vi "DE10_DAQ.vi"() -> ()   [LabVIEW 2014]
uses:
  Control 1.ctl
  <vilib>/Analysis/baseanly.llb/Mean (DBL).vi
  <vilib>/Analysis/NI_AALBase.lvlib
panel:
  in  "IP Address":string="142.90.140.191"
  out "Selected Analog values":dbl(graph)
  out "Logic Mask":T1={"Up"=FALSE, "Down"=TRUE, "Left"=TRUE, "Right"=TRUE, "Halo"=FALSE, "Density"=FALSE, "Total"=FALSE, "HV"=FALSE, "|L-R|"=FALSE, "|U-D|"=TRUE, "|Den-Tot|"=TRUE, "Sum/Tot"=TRUE, "Tot-Sum"=FALSE, "T1 Vac"=FALSE, "T2 Sum"=FALSE, "TNF Sum"=FALSE}
  out "Digital Input":bool[](array[boolean])
  out "Relay Contact output":bool[](array[boolean])
  in  "Analog Parameter Threshold Setting:":string[][](table) caption="Analog Readback values"
  in  "Update Threshold":bool
  in  "Mask Register":T2={"Up"=FALSE, "Down"=TRUE, "Left"=TRUE, "Right"=TRUE, "Halo"=FALSE, "Density"=FALSE, "Total"=FALSE, "HV"=FALSE, "|L-R|"=FALSE, "|U-D|"=TRUE, "|Den-total|"=TRUE, "Sum/Tot"=TRUE, "Tot-Sum"=FALSE, "T1 Vac"=FALSE, "T2 Sum"=FALSE, "TNF Sum"=FALSE}
  in  "Update PCA gain":bool
  in  "Ch7":enum32{"G0", "G1", "G2", "G3"}(radio)
  in  "Ch6":enum32{"G0", "G1", "G2", "G3"}(radio)
  in  "Ch5":enum32{"G0", "G1", "G2", "G3"}(radio)
  in  "Ch4":enum32{"G0", "G1", "G2", "G3"}(radio)
  in  "Ch3":enum32{"G0", "G1", "G2", "G3"}(radio)
  in  "Ch2":enum32{"G0", "G1", "G2", "G3"}(radio)
  in  "Ch1":enum32{"G0", "G1", "G2", "G3"}(radio)
  in  "Ch0":enum32{"G0", "G1", "G2", "G3"}(radio)
  in  "Control Register":T3={"Output Relay"=FALSE, "Not in use"=TRUE, "Ena temp"=TRUE, "PCA Cal"=FALSE}
  in  "flash2conf":bool
  in  "conf2flash":bool
  out "Analog input channel readback - high precision:":string[][](table) caption="Analog Readback values"
  out "Threshold values:":string[][](table) caption="Analog Readback values"
  out "Analog Parameter and Threshold value readback:":T4 caption="Analog Readback values"
  out "Interlock Status":bool[](array[boolean])
  out "Control Register":bool[](array[boolean])
  out "Temperature":dbl(graph)
  out "sFIFO Words":i32=1024
  out "Display channel":u16
  out "Avg (mV)":dbl format="%#_4g"
  out "RMS (mV)":dbl format="%#_4g"
  in  "Waveform\nChannel":T5(radio)
  out "MB Firmware ver:":string="FPGA_VER?"
  out "FPGA ver:":string="FPGA_VER?"
  in  "Enable waveform Acq":bool
  out "Fast FIFO( waveform from selected channel)":dbl[](graph)
  in  "Reg name":string
  out "Read back Value":i32 format="%x"
  in  "Read":bool
  in  "Value to write":i32
  in  "Write":bool
  in  "stop":bool
  in  "PORT":u16=2022
  out "error out":errorcluster
  # "Notes: \n1.) Noise p-p value: measrued on Dec.2,2018:\n40 pA for HG, 10 nA for LG;\n2.) Trancation error gives -0.07 uA for Analog value readback;\nLast updated: January 8,2019 \n3.)Mask bit: check means \"paticipation\""
  # "PCA gain selection:"
  # "Conf EEPROM operation"
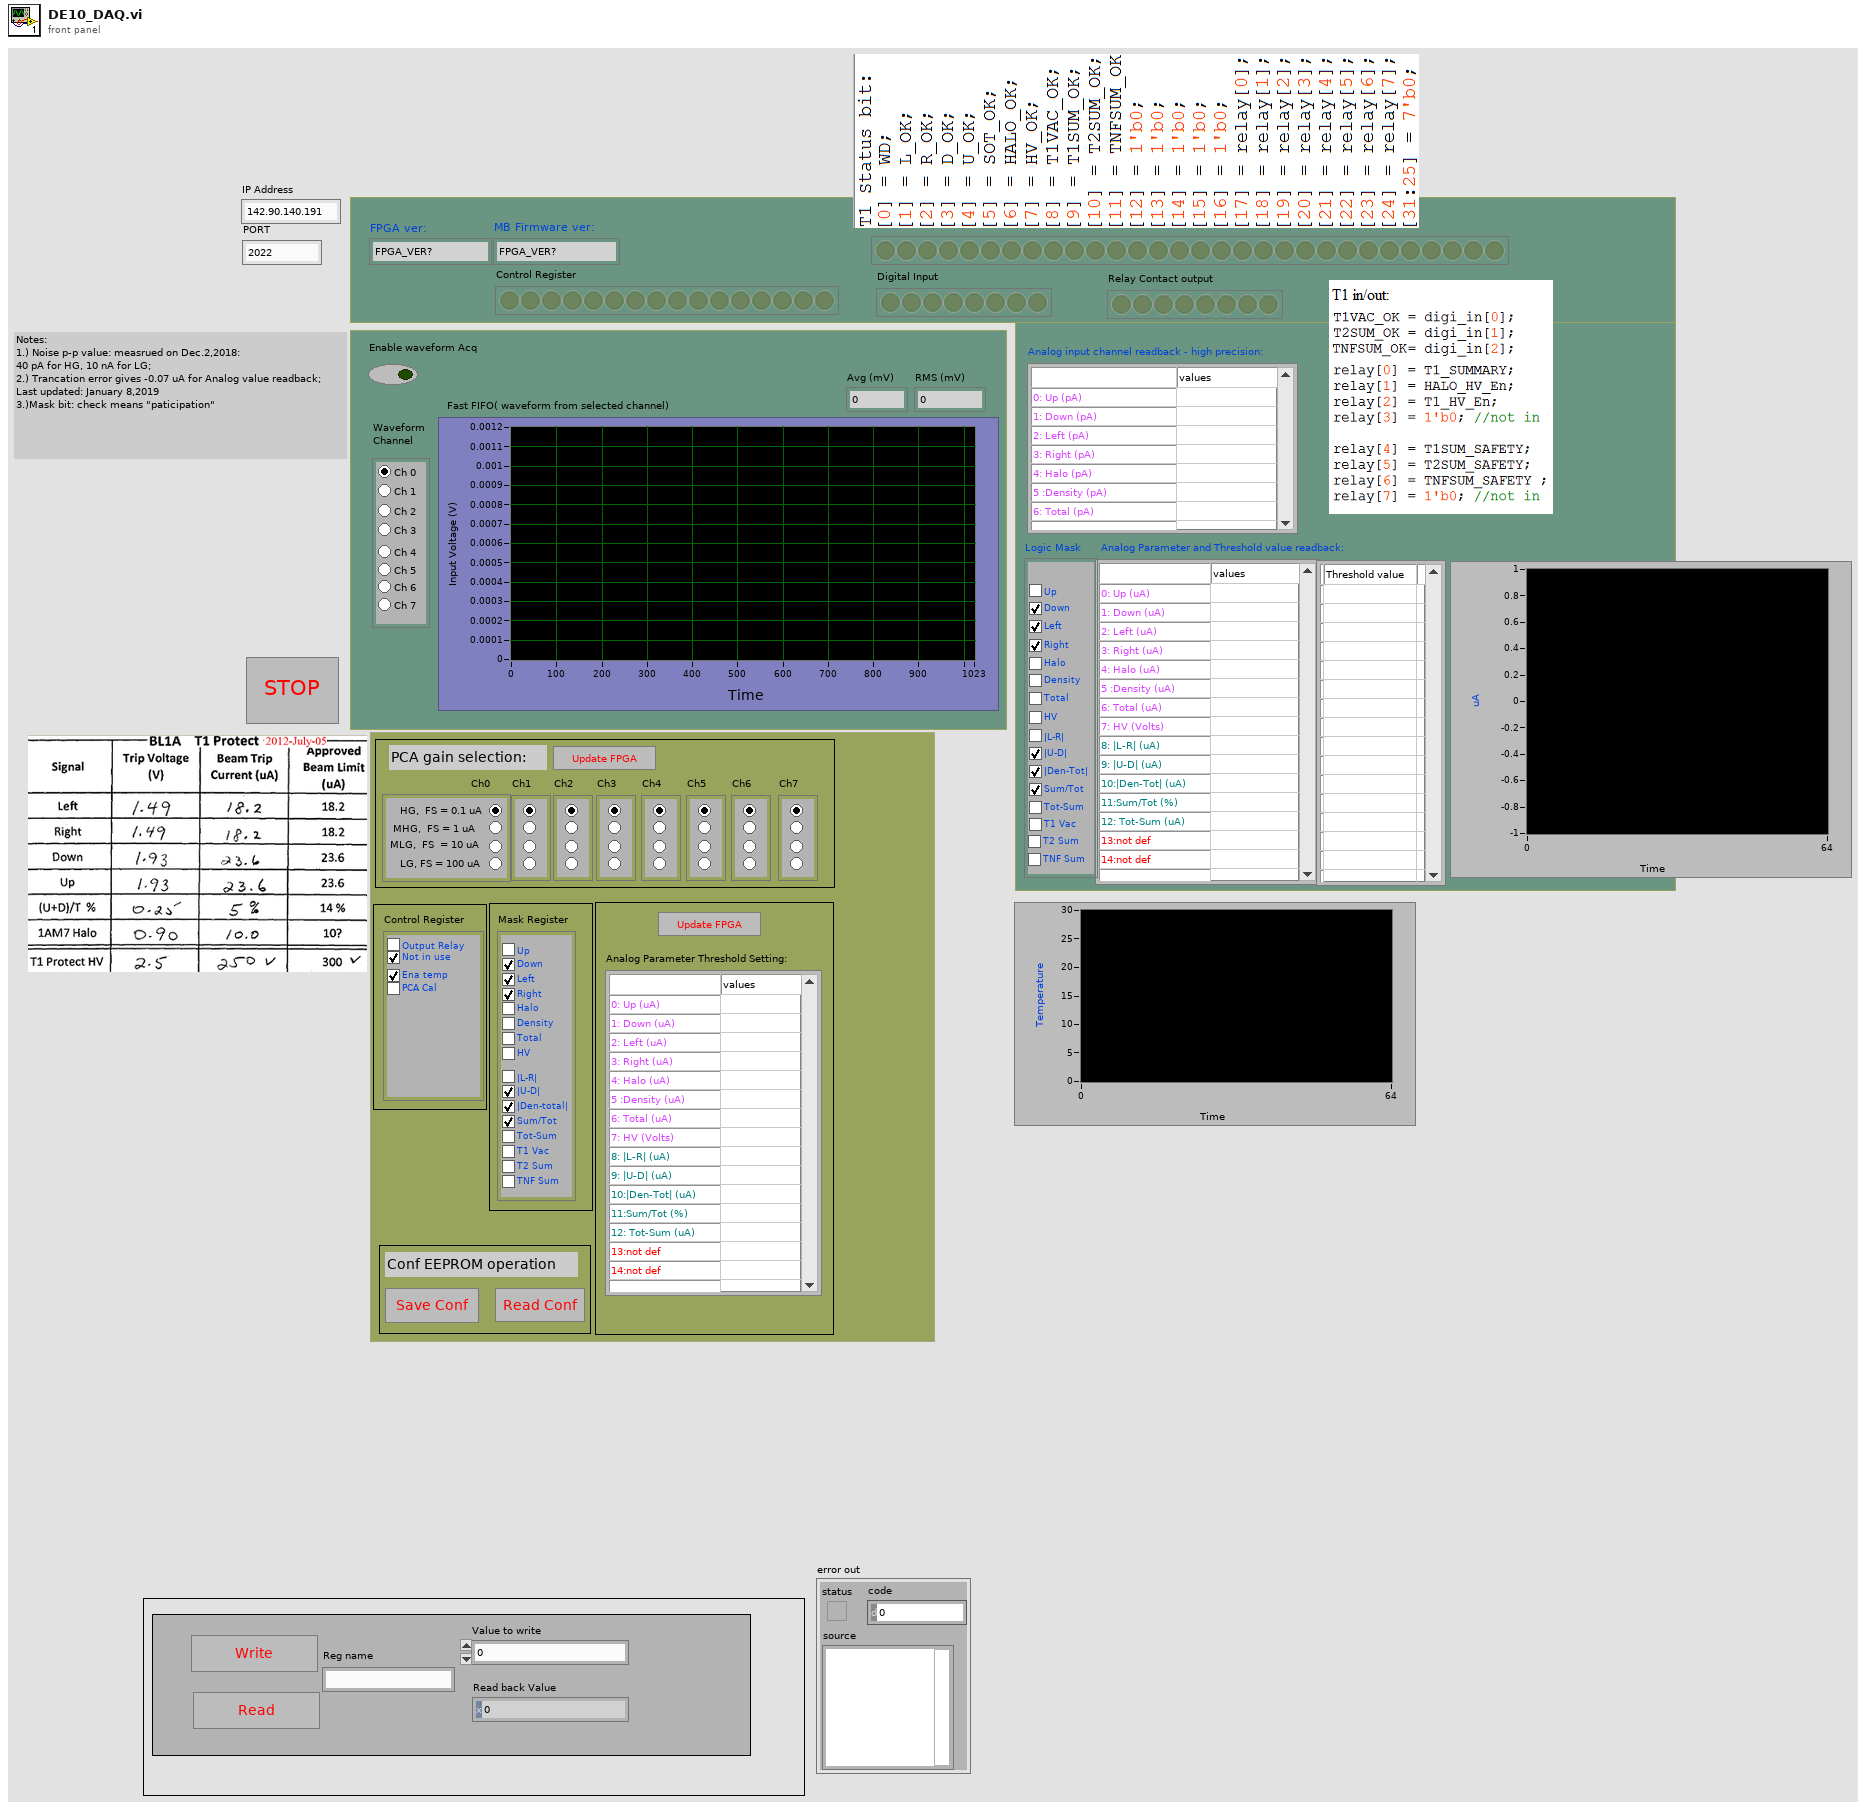
[diagram p1: front panel]
types:
  T1 = cluster{"Up":bool, "Down":bool, "Left":bool, "Right":bool, "Halo":bool, "Density":bool, "Total":bool, "HV":bool, "|L-R|":bool, "|U-D|":bool, "|Den-Tot|":bool, "Sum/Tot":bool, "Tot-Sum":bool, "T1 Vac":bool, "T2 Sum":bool, "TNF Sum":bool}
  T2 = cluster{"Up":bool, "Down":bool, "Left":bool, "Right":bool, "Halo":bool, "Density":bool, "Total":bool, "HV":bool, "|L-R|":bool, "|U-D|":bool, "|Den-total|":bool, "Sum/Tot":bool, "Tot-Sum":bool, "T1 Vac":bool, "T2 Sum":bool, "TNF Sum":bool}
  T3 = cluster{"Output Relay":bool, "Not in use":bool, "Ena temp":bool, "PCA Cal":bool}
  T4 = typedef "Control 1.ctl" = string[][]
  T5 = enum32{"Ch 0", "Ch 1", "Ch 2", "Ch 3", "Ch 4", "Ch 5", "Ch 6", "Ch 7"}
  T6 = cluster{bool, bool, bool, bool, bool, bool, bool, bool, bool, bool, bool, bool, bool, bool, bool, bool}
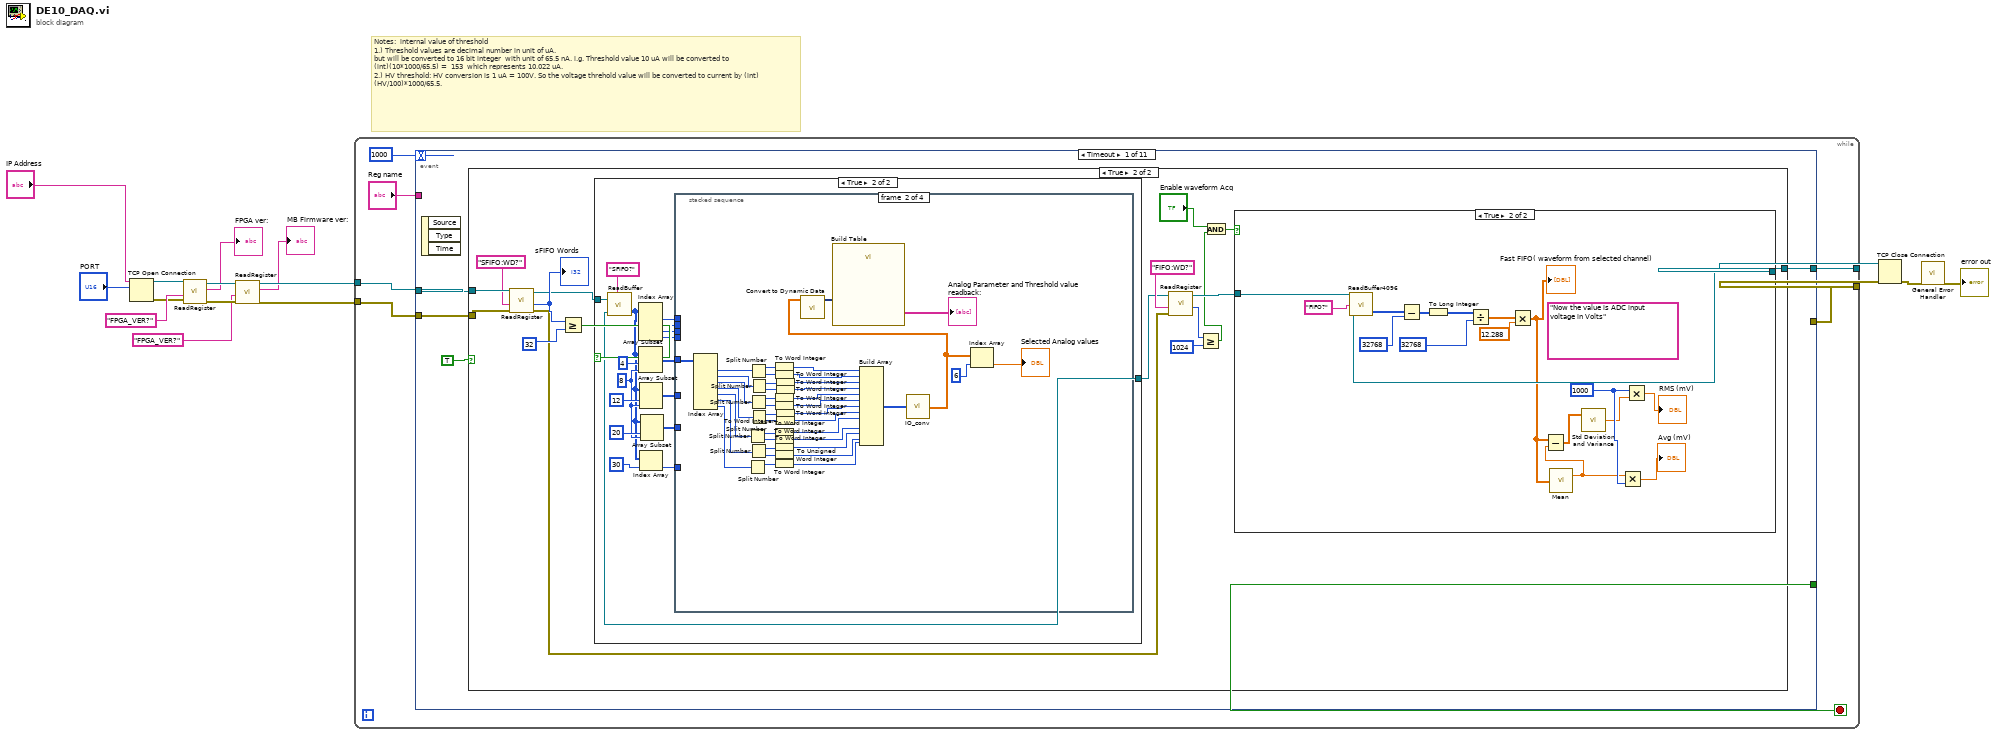
[diagram p0: block diagram]
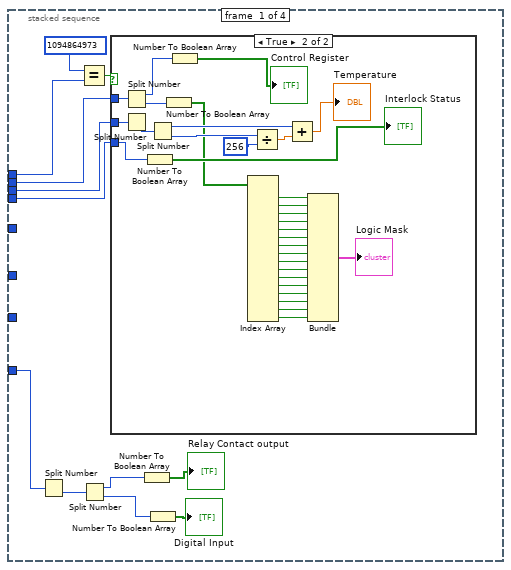
[diagram p4: hidden frame]
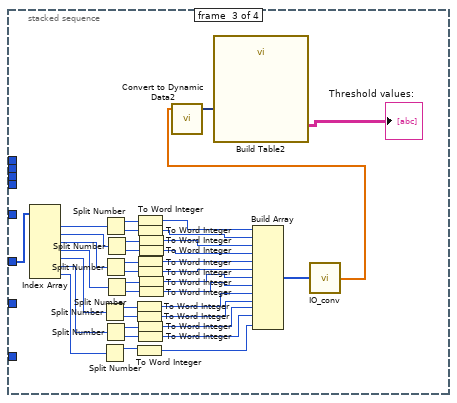
[diagram p6: hidden frame]
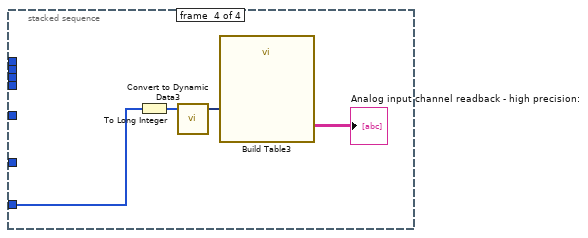
[diagram p7: hidden frame]
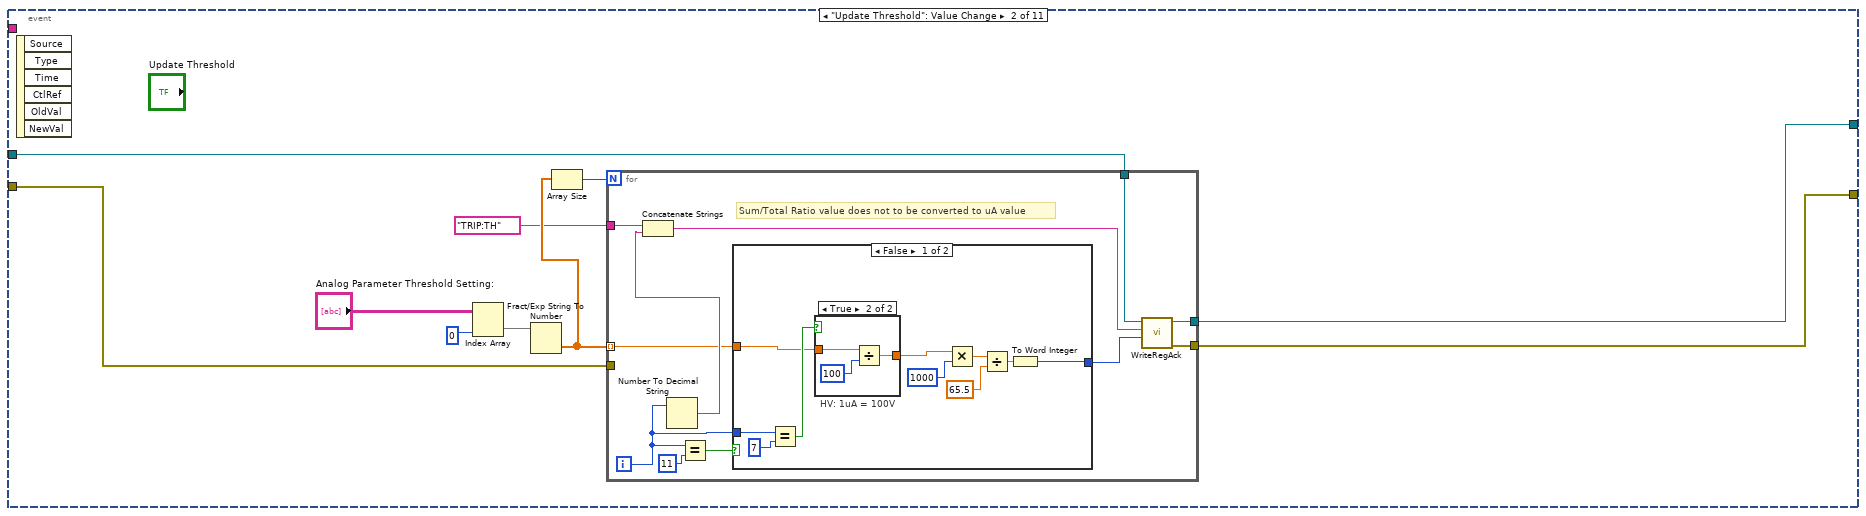
[diagram p9: hidden frame]
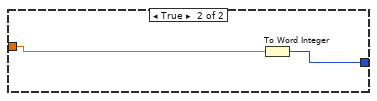
[diagram p11: hidden frame]
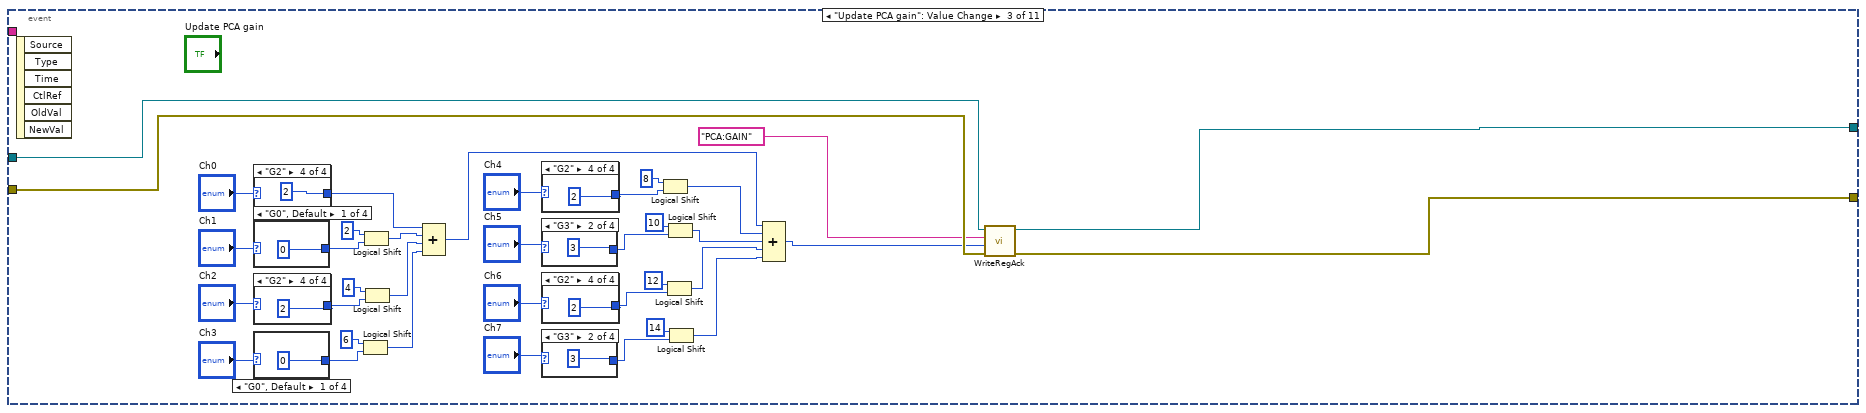
[diagram p12: hidden frame]
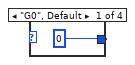
[diagram p13: hidden frame]
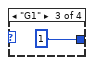
[diagram p14: hidden frame]
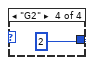
[diagram p15: hidden frame]
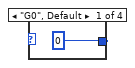
[diagram p16: hidden frame]
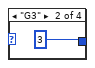
[diagram p17: hidden frame]
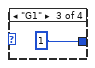
[diagram p18: hidden frame]
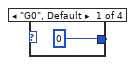
[diagram p19: hidden frame]
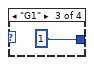
[diagram p20: hidden frame]
diagram:
  # "Notes:  internal value of threshold \n1.) Threshold values are decimal number in unit of uA.\nbut will be converted to 16 bit integer  with unit of 65.5 nA. i.g. Threshold value 10 uA will be converted to (int)(10*1000/65.5) =  153  which represents 10.022 uA. \n2.) HV threshold: HV conversion is 1 uA = 100V. So the voltage threhold value will be converted to current by (int) (HV/100)*1000/65.5."
  n1 = TCP Open Connection(address="IP Address", remote port or service name="PORT") -> (connection ID=w11:refnum<k5>, error out=w7:errorcluster)  [unwired: 3 in]
  n2 = call "ReadRegister.vi"("error in"=w7, "string in"="FPGA_VER?", "connection ID in"=w11) -> ("error out"=w6:errorcluster, "string out"=→"FPGA ver:":string, "connection ID out"=w10:refnum<k5>)  [unwired: 2 in, 2 out]
  n3 = call "ReadRegister.vi"("error in"=w6, "string in"="FPGA_VER?", "connection ID in"=w10) -> ("error out"=w5:errorcluster, "string out"=→"MB Firmware ver:":string, "connection ID out"=w9:refnum<k5>)  [unwired: 2 in, 2 out]
  n4 = while {
    tunnel: [w23] -> w15
    tunnel: [w22] -> w14
    tunnel: w9 -> [w18]
    tunnel: w5 -> [w17]
    stop <- w21 stop-if-true
    n5 = event shown="[0] Timeout" {
      selector: _ -> [_ _ _ _ _ _ _ _ _ _ _]
      dyn-events: _ -> [_ _ _ _ _ _ _ _ _ _ _]
      timeout: 1000 -> [_ _ _ _ _ _ _ _ _ _ _]
      tunnel: w18 -> [w26 w210 w249 w318 w330 w334 w361 w375 w381 w384 w473]
      tunnel: [w27 w208 w247 w316 w327 w333 w356 _ w379 _ w473] -> w23
      tunnel: w17 -> [w25 w209 w248 w317 w329 w331 w360 w373 w377 w385 w472]
      tunnel: [_ w207 w246 w315 w328 w332 w357 w372 w378 _ w472] -> w22
      tunnel: [_ _ _ _ _ _ _ _ _ _ "stop"] -> w21
      tunnel: "Reg name" -> [_ _ _ w313 _ _ _ _ _ _ _]
      tunnel: [_ _ _ _ _ _ _ w371 _ _ _] -> _
      event Timeout {
        n6 = event-data() -> ()  [unwired: 1 in, 3 out]
        n7 = case shown="True" TRUE {
          tunnel: [w28 w45] -> w27
          tunnel: w26 -> [w28 w40]
          tunnel: w25 -> [_ w39]
          frame False {
          }
          frame True {
            n8 = call "ReadRegister.vi"("error in"=w39, "string in"="SFIFO:WD?", "connection ID in"=w40) -> ("error out"=w32:errorcluster, "number out"=w36:i32, "connection ID out"=w34:refnum<k5>)  [unwired: 2 in, 2 out]
            "sFIFO Words" <- w36
            n9 = Greater Or Equal?(x=w36, y=32) -> (x >= y?=w35:bool)
            n10 = case shown="True" w35 {
              tunnel: w34 -> [w46 w62]
              tunnel: [w46 w57] -> w33
              frame False {
              }
              frame True {
                w51 = 8
                n11 = call "ReadBuffer.vi"("string in"="SFIFO?", "connection ID in"=w62) -> ("FIFO32_data"=w48:u32[], "connection ID out"=w57:refnum<k5>)  [unwired: 2 in]
                n12 = Index Array(array=w48) -> (element #1=w61:u32, element #2=w60:u32, element #3=w59:u32, element #4=w58:u32)  [unwired: 4 in]
                n13 = Array Subset(array=w48, index=4, length=w51) -> (w55:u32[])
                n14 = Array Subset(array=w48, index=12, length=w51) -> (w54:u32[])
                n15 = Index Array(array=w48, index=30) -> (element=w47:u32)
                n16 = Array Subset(array=w48, index=20, length=w51) -> (w50:u32[])
                n17 = stacked-sequence {
                  tunnel: w61 -> [w74 _ _ _]
                  tunnel: w60 -> [w72 _ _ _]
                  tunnel: w59 -> [w71 _ _ _]
                  tunnel: w58 -> [w70 _ _ _]
                  tunnel: w55 -> [_ w146 _ _]
                  tunnel: w54 -> [_ _ w151 _]
                  tunnel: w50 -> [_ _ _ w185]
                  tunnel: w47 -> [w69 _ _ _]
                  frame #0 {
                    n18 = Split Number(x=w69) -> (lo(x)=w68:u16)  [unwired: 1 out]
                    n19 = Equal?(x=u32 1094864973, y=w74) -> (x = y?=w73:bool)
                    n20 = Split Number(x=w68) -> (hi(x)=w66:u8, lo(x)=w65:u8)
                    n21 = case shown="True" w73 {
                      tunnel: w72 -> [_ w106]
                      tunnel: w71 -> [_ w99]
                      tunnel: w70 -> [_ w95]
                      frame False {
                      }
                      frame True {
                        n22 = Split Number(x=w106) -> (hi(x)=w101:u16, lo(x)=w105:u16)
                        n23 = Split Number(x=w99) -> (lo(x)=w98:u16)  [unwired: 1 out]
                        n24 = Number To Boolean Array(number=w95) -> (Boolean array=→"Interlock Status":bool[])
                        n25 = Split Number(x=w98) -> (hi(x)=w96:u8, lo(x)=w97:u8)
                        n26 = Number To Boolean Array(number=w105) -> (Boolean array=w76:bool[])
                        n27 = Number To Boolean Array(number=w101) -> (Boolean array=→"Control Register":bool[])
                        n28 = Index Array(array=w76) -> (element #1=w77:bool, element #2=w78:bool, element #3=w79:bool, element #4=w80:bool, element #5=w81:bool, element #6=w82:bool, element #7=w83:bool, element #8=w84:bool, element #9=w85:bool, element #10=w86:bool, element #11=w87:bool, element #12=w88:bool, element #13=w89:bool, element #14=w90:bool, element #15=w91:bool, element #16=w92:bool)  [unwired: 16 in]
                        n29 = Divide(x=w97, y=256) -> (x/y=w103:dbl)
                        n30 = Add(x=w96, y=w103) -> (x+y=→"Temperature":dbl)
                        n31 = Bundle(w77, w78, w79, w80, w81, w82, w83, w84, w85, w86, w87, w88, w89, w90, w91, w92) -> (→"Logic Mask":T6)  [unwired: 1 in]
                      }
                    }
                    n32 = Number To Boolean Array(number=w66) -> (Boolean array=→"Relay Contact output":bool[])
                    n33 = Number To Boolean Array(number=w65) -> (Boolean array=→"Digital Input":bool[])
                  }
                  frame #1 {
                    n34 = Index Array(array=w146) -> (element #1=w145:u32, element #2=w136:u32, element #3=w135:u32, element #4=w134:u32, element #5=w129:u32, element #6=w128:u32, element #7=w127:u32)  [unwired: 7 in]
                    n35 = Split Number(x=w129) -> (hi(x)=w133:u16, lo(x)=w132:u16)
                    n36 = Split Number(x=w127) -> (hi(x)=w111:u16)  [unwired: 1 out]
                    n37 = Split Number(x=w145) -> (hi(x)=w144:u16, lo(x)=w143:u16)
                    n38 = Split Number(x=w135) -> (hi(x)=w140:u16, lo(x)=w139:u16)
                    n39 = Split Number(x=w128) -> (hi(x)=w131:u16, lo(x)=w130:u16)
                    n40 = Split Number(x=w136) -> (hi(x)=w142:u16, lo(x)=w141:u16)
                    n41 = Split Number(x=w134) -> (hi(x)=w138:u16, lo(x)=w137:u16)
                    n42 = To Word Integer(number=w133) -> (16bit integer=w118:i16)
                    n43 = To Word Integer(number=w132) -> (16bit integer=w117:i16)
                    n44 = To Word Integer(number=w111) -> (16bit integer=w112:i16)
                    n45 = To Word Integer(number=w144) -> (16bit integer=w126:i16)
                    n46 = To Word Integer(number=w143) -> (16bit integer=w119:i16)
                    n47 = To Word Integer(number=w140) -> (16bit integer=w123:i16)
                    n48 = To Word Integer(number=w139) -> (16bit integer=w122:i16)
                    n49 = To Word Integer(number=w131) -> (16bit integer=w116:i16)
                    n50 = To Unsigned Word Integer(number=w130) -> (unsigned 16bit integer=w115:u16)
                    n51 = To Word Integer(number=w142) -> (16bit integer=w125:i16)
                    n52 = To Word Integer(number=w141) -> (16bit integer=w124:i16)
                    n53 = To Word Integer(number=w138) -> (16bit integer=w121:i16)
                    n54 = To Word Integer(number=w137) -> (16bit integer=w120:i16)
                    n55 = Build Array(w126, w119, w125, w124, w123, w122, w121, w120, w118, w117, w116, w115, w112) -> (w110:u16[])
                    n56 = call "IO_conv.vi"("input"=w110) -> ("output"=w109:dbl[])
                    n57 = call "Convert to Dynamic Data"("Array"=w109) -> ("Dynamic Data Type"=w114:dynamicdata)  [unwired: 3 in]
                    n58 = call "Build Table"("Signals"=w114) -> ("Table"=→"Analog Parameter and Threshold value readback:":string[][])  [unwired: 9 in, 1 out]
                    n59 = Index Array(array=w109, index=6) -> (element=→"Selected Analog values":dbl)
                  }
                  frame #2 {
                    n60 = Index Array(array=w151) -> (element #1=w183:u32, element #2=w174:u32, element #3=w173:u32, element #4=w172:u32, element #5=w167:u32, element #6=w166:u32, element #7=w165:u32)  [unwired: 7 in]
                    n61 = Split Number(x=w167) -> (hi(x)=w171:u16, lo(x)=w170:u16)
                    n62 = Split Number(x=w165) -> (hi(x)=w149:u16)  [unwired: 1 out]
                    n63 = Split Number(x=w183) -> (hi(x)=w182:u16, lo(x)=w181:u16)
                    n64 = Split Number(x=w173) -> (hi(x)=w178:u16, lo(x)=w177:u16)
                    n65 = Split Number(x=w166) -> (hi(x)=w169:u16, lo(x)=w168:u16)
                    n66 = Split Number(x=w174) -> (hi(x)=w180:u16, lo(x)=w179:u16)
                    n67 = Split Number(x=w172) -> (hi(x)=w176:u16, lo(x)=w175:u16)
                    n68 = To Word Integer(number=w171) -> (16bit integer=w156:i16)
                    n69 = To Word Integer(number=w170) -> (16bit integer=w155:i16)
                    n70 = To Word Integer(number=w149) -> (16bit integer=w152:i16)
                    n71 = To Word Integer(number=w182) -> (16bit integer=w164:i16)
                    n72 = To Word Integer(number=w181) -> (16bit integer=w157:i16)
                    n73 = To Word Integer(number=w178) -> (16bit integer=w161:i16)
                    n74 = To Word Integer(number=w177) -> (16bit integer=w160:i16)
                    n75 = To Word Integer(number=w169) -> (16bit integer=w154:i16)
                    n76 = To Word Integer(number=w168) -> (16bit integer=w153:i16)
                    n77 = To Word Integer(number=w180) -> (16bit integer=w163:i16)
                    n78 = To Word Integer(number=w179) -> (16bit integer=w162:i16)
                    n79 = To Word Integer(number=w176) -> (16bit integer=w159:i16)
                    n80 = To Word Integer(number=w175) -> (16bit integer=w158:i16)
                    n81 = Build Array(w164, w157, w163, w162, w161, w160, w159, w158, w156, w155, w154, w153, w152) -> (w148:i16[])
                    n82 = call "IO_conv.vi"("input"=w148) -> ("output"=w147:dbl[])
                    n83 = call "Convert to Dynamic Data2"("Array"=w147) -> ("Dynamic Data Type"=w184:dynamicdata)  [unwired: 3 in]
                    n84 = call "Build Table2"("Signals"=w184) -> ("Table"=→"Threshold values:":string[][])  [unwired: 9 in, 1 out]
                  }
                  frame #3 {
                    n85 = To Long Integer(number=w185) -> (32bit integer=w186:i32[])
                    n86 = call "Convert to Dynamic Data3"("Array"=w186) -> ("Dynamic Data Type"=w188:dynamicdata)  [unwired: 3 in]
                    n87 = call "Build Table3"("Signals"=w188) -> ("Table"=→"Analog input channel readback - high precision:":string[][])  [unwired: 9 in, 1 out]
                  }
                }
              }
            }
            n88 = call "ReadRegister.vi"("error in"=w32, "string in"="FIFO:WD?", "connection ID in"=w33) -> ("number out"=w41:i32, "connection ID out"=w44:refnum<k5>)  [unwired: 2 in, 3 out]
            n89 = Greater Or Equal?(x=w41, y=1024) -> (x >= y?=w29:bool)
            n90 = And(x="Enable waveform Acq", y=w29) -> (x .and. y?=w30:bool)
            n91 = case shown="True" w30 {
              tunnel: [w189 w206] -> w45
              tunnel: w44 -> [w189 w205]
              frame False {
              }
              frame True {
                w195 = 1000
                (unwired) "Now the value is ADC input voltage in Volts"
                n92 = call "ReadBuffer4096.vi"("string in"="FIFO?", "connection ID in"=w205) -> ("FIFO32_data"=w200:u32[], "connection ID out"=w206:refnum<k5>)  [unwired: 2 in]
                n93 = Subtract(x=w200, y=32768) -> (x-y=w197:u32[])
                n94 = To Long Integer(number=w197) -> (32bit integer=w198:i32[])
                n95 = Divide(x=w198, y=32768) -> (x/y=w199:dbl[])
                n96 = Multiply(x=w199, y=12.288) -> (x*y=w191:dbl[])
                "Fast FIFO( waveform from selected channel)" <- w191
                n97 = call-poly <vilib>:"Mean.vi"("X"=w191) -> ("mean"=w192:dbl)  [unwired: 1 out]
                n98 = Subtract(x=w191, y=w192) -> (x-y=w190:dbl[])
                n99 = call <vilib>:"Std Deviation and Variance.vi"("X"=w190) -> ("standard deviation"=w194:dbl)  [unwired: 1 in, 2 out]
                n100 = Multiply(x=w192, y=w195) -> (x*y=→"Avg (mV)":dbl)
                n101 = Multiply(x=w195, y=w194) -> (x*y=→"RMS (mV)":dbl)
              }
            }
          }
        }
      }
      event "Update Threshold": Value Change {
        n102 = event-data() -> ()  [unwired: 1 in, 6 out]
        n103 = Index Array(array="Analog Parameter Threshold Setting:", index (col)=0) -> (element=w215:string[])  [unwired: 1 in]
        n104 = Fract/Exp String To Number(string=w215) -> (number=w212:dbl[])  [unwired: 3 in, 1 out]
        n105 = Array Size(array=w212) -> (size(s)=w213:i32)
        n106 = for {
          N: w213 -> [_]
          tunnel: w212 -> [w221] mode=indexing
          tunnel: "TRIP:TH" -> [w227]
          tunnel: w210 -> [w224]
          tunnel: w209 -> [_]
          tunnel: [w223] -> w208
          tunnel: [w222] -> w207
          i -> [w218]
          # "Sum/Total Ratio value does not to be converted to uA value"
          n107 = Number To Decimal String(number=w218) -> (decimal integer string=w226:string)  [unwired: 1 in]
          n108 = Concatenate Strings(w227, w226) -> (w225:string)
          n109 = Equal?(x=w218, y=11) -> (x = y?=w219:bool)
          n110 = case shown="False" w219 {
            tunnel: w218 -> [w229 _]
            tunnel: w221 -> [w230 w242]
            tunnel: [w228 w243] -> w220
            frame False {
              n111 = Equal?(x=w229, y=7) -> (x = y?=w231:bool)
              n112 = case "HV: 1uA = 100V" shown="True" w231 {
                tunnel: w230 -> [w238 w241]
                tunnel: [w238 w239] -> w233
                frame False {
                }
                frame True {
                  n113 = Divide(x=w241, y=100) -> (x/y=w239:dbl)
                }
              }
              n114 = Multiply(x=w233, y=1000) -> (x*y=w235:dbl)
              n115 = Divide(x=w235, y=65.5) -> (x/y=w237:dbl)
              n116 = To Word Integer(number=w237) -> (16bit integer=w228:i16)
            }
            frame True {
              n117 = To Word Integer(number=w242) -> (16bit integer=w243:i16)
            }
          }
          n118 = call "WriteRegAck.vi"("value in"=w220, "string in"=w225, "connection ID in"=w224) -> ("error out"=w222:errorcluster, "connection ID out"=w223:refnum<k5>)  [unwired: 2 in, 3 out]
        }
      }
      event "Update PCA gain": Value Change {
        n119 = event-data() -> ()  [unwired: 1 in, 6 out]
        n120 = case shown="\"G2\"" "Ch0" {
          tunnel: [0 3 1 2] -> w258
          frame "G0", Default {
          }
          frame "G3" {
          }
          frame "G1" {
          }
          frame "G2" {
          }
        }
        n121 = case shown="\"G0\", Default" "Ch1" {
          tunnel: [0 3 1 2] -> w271
          frame "G0", Default {
          }
          frame "G3" {
          }
          frame "G1" {
          }
          frame "G2" {
          }
        }
        n122 = case shown="\"G2\"" "Ch2" {
          tunnel: [0 3 1 2] -> w260
          frame "G0", Default {
          }
          frame "G3" {
          }
          frame "G1" {
          }
          frame "G2" {
          }
        }
        n123 = case shown="\"G0\", Default" "Ch3" {
          tunnel: [0 3 1 2] -> w259
          frame "G0", Default {
          }
          frame "G3" {
          }
          frame "G1" {
          }
          frame "G2" {
          }
        }
        n124 = Logical Shift(y=6, x=w259) -> (x << y=w255:i32)
        n125 = Logical Shift(y=2, x=w271) -> (x << y=w257:i32)
        n126 = Logical Shift(y=4, x=w260) -> (x << y=w256:i32)
        n127 = Compound Arithmetic op=ADD(w258, w257, w256, w255) -> (w254:i32)
        n128 = case shown="\"G2\"" "Ch4" {
          tunnel: [0 3 1 2] -> w264
          frame "G0", Default {
          }
          frame "G3" {
          }
          frame "G1" {
          }
          frame "G2" {
          }
        }
        n129 = case shown="\"G3\"" "Ch5" {
          tunnel: [0 3 1 2] -> w263
          frame "G0", Default {
          }
          frame "G3" {
          }
          frame "G1" {
          }
          frame "G2" {
          }
        }
        n130 = case shown="\"G2\"" "Ch6" {
          tunnel: [0 3 1 2] -> w262
          frame "G0", Default {
          }
          frame "G3" {
          }
          frame "G1" {
          }
          frame "G2" {
          }
        }
        n131 = case shown="\"G3\"" "Ch7" {
          tunnel: [0 3 1 2] -> w261
          frame "G0", Default {
          }
          frame "G3" {
          }
          frame "G1" {
          }
          frame "G2" {
          }
        }
        n132 = Logical Shift(y=8, x=w264) -> (x << y=w253:i32)
        n133 = Logical Shift(y=12, x=w262) -> (x << y=w251:i32)
        n134 = Logical Shift(y=10, x=w263) -> (x << y=w252:i32)
        n135 = Logical Shift(y=14, x=w261) -> (x << y=w250:i32)
        n136 = Compound Arithmetic op=ADD(w254, w253, w252, w251, w250) -> (w244:i32)
        n137 = call "WriteRegAck.vi"("error in"=w248, "value in"=w244, "string in"="PCA:GAIN", "connection ID in"=w249) -> ("error out"=w246:errorcluster, "connection ID out"=w247:refnum<k5>)  [unwired: 1 in, 3 out]
      }
      event "Write": Value Change {
        n138 = event-data() -> ()  [unwired: 1 in, 6 out]
        n139 = call "WriteRegAck.vi"("error in"=w317, "value in"="Value to write", "string in"=w313, "connection ID in"=w318) -> ("error out"=w315:errorcluster, "connection ID out"=w316:refnum<k5>)  [unwired: 1 in, 3 out]
      }
      event "Control Register": Value Change {
        n140 = event-data() -> ()  [unwired: 1 in, 6 out]
        n141 = Unbundle By Name("Control Register") -> ("Output Relay"=w319:bool, "Ena temp"=w322:bool, "PCA Cal"=w321:bool)  [unwired: 1 out]
        n142 = Build Array(w319, FALSE, w322, w321) -> (w325:bool[])
        n143 = Boolean Array To Number(Boolean array=w325) -> (number=w324:u32)
        n144 = call "WriteRegAck.vi"("error in"=w329, "value in"=w324, "string in"="CR", "connection ID in"=w330) -> ("error out"=w328:errorcluster, "connection ID out"=w327:refnum<k5>)  [unwired: 1 in, 3 out]
      }
      event "Mask Register": Value Change {
        n145 = event-data() -> ()  [unwired: 1 in, 6 out]
        n146 = Unbundle By Name("Mask Register") -> ("Up"=w352:bool, "Down"=w351:bool, "Left"=w350:bool, "Right"=w349:bool, "Halo"=w348:bool, "Density"=w347:bool, "Total"=w346:bool, "HV"=w345:bool, "|L-R|"=w344:bool, "|U-D|"=w343:bool, "|Den-total|"=w342:bool, "Sum/Tot"=w341:bool, "Tot-Sum"=w340:bool, "T1 Vac"=w339:bool, "T2 Sum"=w338:bool, "TNF Sum"=w337:bool)
        n147 = Build Array(w352, w351, w350, w349, w348, w347, w346, w345, w344, w343, w342, w341, w340, w339, w338, w337) -> (w353:bool[])
        n148 = Boolean Array To Number(Boolean array=w353) -> (number=w335:u32)
        n149 = call "WriteRegAck.vi"("error in"=w331, "value in"=w335, "string in"="MR", "connection ID in"=w334) -> ("error out"=w332:errorcluster, "connection ID out"=w333:refnum<k5>)  [unwired: 1 in, 3 out]
      }
      event "Waveform\nChannel": Value Change {
        n150 = event-data() -> ()  [unwired: 1 in, 6 out]
        n151 = case shown="\"Ch 0\", Default" "Waveform\nChannel" {
          tunnel: [0 4 5 6 7 1 2 3] -> w355
          frame "Ch 0", Default {
          }
          frame "Ch 4" {
          }
          frame "Ch 5" {
          }
          frame "Ch 6" {
          }
          frame "Ch 7" {
          }
          frame "Ch 1" {
          }
          frame "Ch 2" {
          }
          frame "Ch 3" {
          }
        }
        "Display channel" <- w355
        n152 = call "WriteRegAck.vi"("error in"=w360, "value in"=w355, "string in"="CH:SEL", "connection ID in"=w361) -> ("error out"=w357:errorcluster, "connection ID out"=w356:refnum<k5>)  [unwired: 1 in, 3 out]
      }
      event "Read": Value Change {
        n153 = event-data() -> ()  [unwired: 1 in, 6 out]
        n154 = call "ReadRegister.vi"("error in"=w373, "string in"="TRIP:TH4?", "connection ID in"=w375) -> ("error out"=w372:errorcluster, "number out"=→"Read back Value":i32, "connection ID out"=w371:refnum<k5>)  [unwired: 2 in, 2 out]
      }
      event "conf2flash": Value Change {
        n155 = event-data() -> ()  [unwired: 1 in, 6 out]
        n156 = call "WriteRegAck.vi"("error in"=w377, "value in"=0, "string in"="CONF2EEPROM", "connection ID in"=w381) -> ("error out"=w378:errorcluster, "connection ID out"=w379:refnum<k5>)  [unwired: 1 in, 3 out]
      }
      event "flash2conf": Value Change {
        n157 = event-data() -> ()  [unwired: 1 in, 6 out]
        n158 = call "WriteRegAck.vi"("error in"=w385, "value in"=0, "string in"="EEPROM2CONF", "connection ID in"=w384) -> ("error out"=w382:errorcluster, "connection ID out"=w383:refnum<k5>)  [unwired: 1 in, 3 out]
        n159 = stacked-sequence {
          tunnel: w383 -> [_ w397 w413 w453 w462 _]
          tunnel: w382 -> [_ w395 w412 w452 w461 _]
          frame #0 {
            n160 = Wait (ms)(milliseconds to wait=500) -> ()  [unwired: 1 out]
          }
          frame #1 {
            n161 = call "ReadRegister.vi"("error in"=w395, "string in"="CR?", "connection ID in"=w397) -> ("boolean array out"=w389:bool[])  [unwired: 2 in, 4 out]
            n162 = Index Array(array=w389) -> (element #1=w394:bool, element #2=w393:bool, element #3=w392:bool, element #4=w391:bool)  [unwired: 4 in]
            n163 = local write "Control Register"(w389) -> ()
            n164 = Bundle(w394, w393, w392, w391) -> (w390:cluster{bool, bool, bool, bool})  [unwired: 1 in]
            n165 = local write "Control Register"(w390) -> ()
          }
          frame #2 {
            n166 = call "ReadRegister.vi"("error in"=w412, "string in"="MR?", "connection ID in"=w413) -> ("boolean array out"=w398:bool[])  [unwired: 2 in, 4 out]
            n167 = Index Array(array=w398) -> (element #1=w417:bool, element #2=w416:bool, element #3=w415:bool, element #4=w414:bool, element #5=w411:bool, element #6=w410:bool, element #7=w409:bool, element #8=w408:bool, element #9=w407:bool, element #10=w406:bool, element #11=w405:bool, element #12=w404:bool, element #13=w403:bool, element #14=w402:bool, element #15=w401:bool, element #16=w400:bool)  [unwired: 16 in]
            n168 = Bundle(w417, w416, w415, w414, w411, w410, w409, w408, w407, w406, w405, w404, w403, w402, w401, w400) -> (w399:T6)  [unwired: 1 in]
            n169 = local write "Mask Register"(w399) -> ()
          }
          frame #3 {
            n170 = call "ReadRegister.vi"("error in"=w452, "string in"="PCA:GAIN?", "connection ID in"=w453) -> ("boolean array out"=w451:bool[])  [unwired: 2 in, 4 out]
            n171 = Index Array(array=w451) -> (element #1=w450:bool, element #2=w449:bool, element #3=w445:bool, element #4=w444:bool, element #5=w440:bool, element #6=w439:bool, element #7=w438:bool, element #8=w437:bool, element #9=w434:bool, element #10=w433:bool, element #11=w432:bool, element #12=w431:bool, element #13=w428:bool, element #14=w427:bool, element #15=w426:bool, element #16=w425:bool)  [unwired: 16 in]
            n172 = Build Array(w450, w449) -> (w448:bool[])
            n173 = Build Array(w445, w444) -> (w446:bool[])
            n174 = Build Array(w440, w439) -> (w442:bool[])
            n175 = Build Array(w438, w437) -> (w441:bool[])
            n176 = Build Array(w434, w433) -> (w436:bool[])
            n177 = Build Array(w432, w431) -> (w435:bool[])
            n178 = Build Array(w428, w427) -> (w430:bool[])
            n179 = Build Array(w426, w425) -> (w429:bool[])
            n180 = Boolean Array To Number(Boolean array=w448) -> (number=w447:u32)
            n181 = Boolean Array To Number(Boolean array=w442) -> (number=w424:u32)
            n182 = Boolean Array To Number(Boolean array=w436) -> (number=w422:u32)
            n183 = Boolean Array To Number(Boolean array=w430) -> (number=w420:u32)
            n184 = Boolean Array To Number(Boolean array=w446) -> (number=w443:u32)
            n185 = Boolean Array To Number(Boolean array=w441) -> (number=w423:u32)
            n186 = Boolean Array To Number(Boolean array=w435) -> (number=w421:u32)
            n187 = Boolean Array To Number(Boolean array=w429) -> (number=w419:u32)
            n188 = local write "Ch1"(w443) -> ()
            n189 = local write "Ch0"(w447) -> ()
            n190 = local write "Ch4"(w422) -> ()
            n191 = local write "Ch6"(w420) -> ()
            n192 = local write "Ch7"(w419) -> ()
            n193 = local write "Ch2"(w424) -> ()
            n194 = local write "Ch3"(w423) -> ()
            n195 = local write "Ch5"(w421) -> ()
          }
          frame #4 {
            n196 = for {
              N: 13 -> [_]
              tunnel: w462 -> [w471]
              tunnel: w461 -> [w470]
              tunnel: [w468] -> w456 mode=indexing
              tunnel: "TRIP:TH" -> [w467]
              i -> [w466]
              n197 = Number To Decimal String(number=w466) -> (decimal integer string=w465:string)  [unwired: 1 in]
              n198 = Concatenate Strings(w467, w465, "?") -> (w463:string)
              n199 = call "ReadRegister.vi"("error in"=w470, "string in"=w463, "connection ID in"=w471) -> ("number out"=w469:i32)  [unwired: 2 in, 4 out]
              n200 = Split Number(x=w469) -> (lo(x)=w468:u16)  [unwired: 1 out]
            }
            n201 = call "IO_conv.vi"("input"=w456) -> ("output"=w455:dbl[])
            n202 = call "Convert to Dynamic Data4"("Array"=w455) -> ("Dynamic Data Type"=w458:dynamicdata)  [unwired: 3 in]
            n203 = call "Build Table4"("Signals"=w458) -> ("Table"=w457:string[][])  [unwired: 9 in, 1 out]
            n204 = local write "Analog Parameter Threshold Setting:"(w457) -> ()
          }
          frame #5 {
          }
        }
      }
      event "stop": Value Change {
        n205 = event-data() -> ()  [unwired: 1 in, 6 out]
      }
    }
  }
  n206 = TCP Close Connection(connection ID=w15, error in (no error)=w14) -> (error out=w13:errorcluster)  [unwired: 1 in, 1 out]
  n207 = call <vilib>:"General Error Handler.vi"("error in (no error)"=w13) -> ("error out"=→"error out":errorcluster)  [unwired: 10 in, 4 out]
